vi "lvmcp_events.vi"() -> ()   [LabVIEW 2015]
uses:
  <vilib>/event_ctls.llb/lveventtype.ctl
panel:
  in  "reference":refnum<vi>
  out "reference out":refnum<vi>
  out "error out":errorcluster
  in  "Dynamic Events":T2(array[cluster])
  in  "Static Control Events":T3(array[cluster])
  in  "Static App/VI Events":T4(array[cluster])
  in  "Frame Index":i32
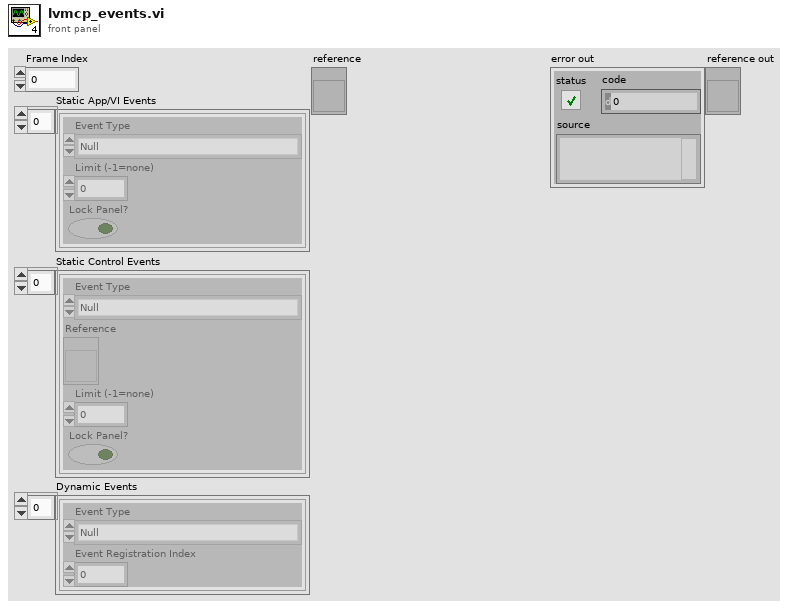
[diagram p1: front panel]
types:
  T1 = typedef "lveventtype.ctl" = enum32{"Null", "Timeout", "Annotation Menu Selection", "Annotation Menu Selection?", "App Instance Close", "App Instance Close?", "Autoscale Range Change", "Bookmark Info Change", "Cell Edit", "Cell Edit?", "Cursor Grab", "Cursor Grab?", "Cursor Menu Selection", "Cursor Menu Selection?", "Cursor Move", "Cursor Release", "Data Change", "Direction Change", "Display State Change", "Drag Ended", "Drag Enter", "Drag Leave", "Drag Over", "Drag Source Update", "Drag Starting", "Drag Starting?", "Drop", "Exec State Change", "Key Down", "Key Down?", "Key Repeat", "Key Repeat?", "Key Up", "Listbox Double Click", "Menu Activation?", "Menu Selection (App)", "Menu Selection? (App)", "Menu Selection (User)", "Mouse Down", "Mouse Down?", "Mouse Enter", "Mouse Leave", "Mouse Move", "Mouse Up", "Mouse Wheel", "NI Security User Change (App)", "Pane Size", "Panel Close", "Panel Close?", "Panel Resize", "Plot Attribute Change", "Scale Range Change", "Shortcut Menu Activation?", "Shortcut Menu Selection (App)", "Shortcut Menu Selection? (App)", "Shortcut Menu Selection (User)", "Tree Double Click", "Tree Drag", "Tree Drag?", "Tree Drop", "Tree Drop?", "Tree Item Close", "Tree Item Close?", "Tree Item Open", "Tree Item Open?", "URL Change?", "User Event", "Value Change"}
  T2 = cluster{"Event Type":T1, "Event Registration Index":i32}[]
  T3 = cluster{"Event Type":T1, "Reference":refnum<vi>, "Limit (-1=none)":i32, "Lock Panel?":bool}[]
  T4 = cluster{"Event Type":T1, "Limit (-1=none)":i32, "Lock Panel?":bool}[]
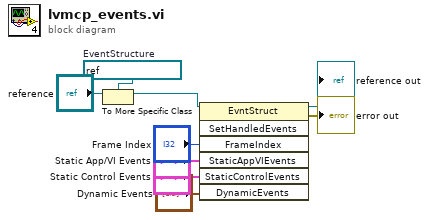
[diagram p0: block diagram]
diagram:
  w9 = refnum<vi> refnum  # EventStructure
  n1 = To More Specific Class(target class=w9, reference="reference") -> (specific class reference=w8:refnum<vi>)  [unwired: 1 in, 1 out]
  n2 = invoke class="EvntStruct" method="SetHandledEvents"(reference=w8, "FrameIndex"="Frame Index", "StaticAppVIEvents"="Static App/VI Events", "StaticControlEvents"="Static Control Events", "DynamicEvents"="Dynamic Events") -> (reference out=→"reference out":refnum<vi>, error out=→"error out":errorcluster)  [unwired: 2 in, 5 out]
